vi "local_roll.vi"() -> (3 "number":i32)   [LabVIEW 2026]
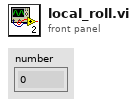
[diagram p1: front panel]
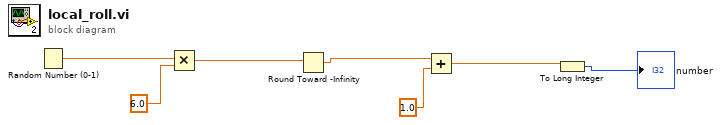
[diagram p0: block diagram]
diagram:
  n1 = Random Number (0-1)() -> (number: 0 to 1=w7:dbl)
  n2 = Multiply(x=w7, y=6.0) -> (x*y=w5:dbl)
  n3 = Round Toward -Infinity(1:w5) -> (0:w4:dbl)
  n4 = Add(x=w4, y=1.0) -> (x+y=w2:dbl)
  n5 = To Long Integer(number=w2) -> (32bit integer=→"number":i32)
